vi "numbe_estimation.vi"(8 "桁数":i32=4, 11 "数値":i32) -> (3 "数値文字列":string)   [LabVIEW 2018]
panel:
  out "文字列":string
  out "配列":string[](array[string])
  out "10進数整数文字列":string
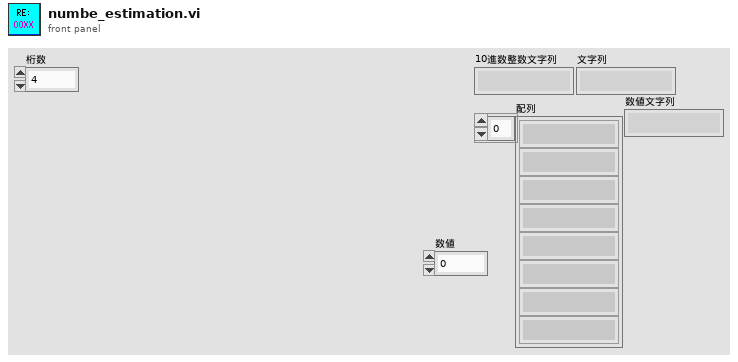
[diagram p1: front panel]
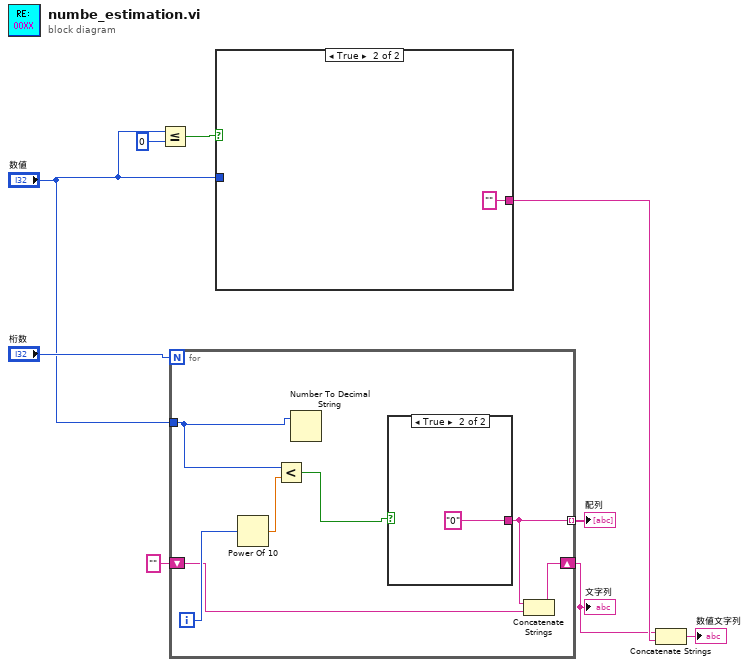
[diagram p0: block diagram]
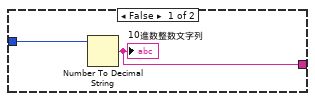
[diagram p2: hidden frame]
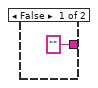
[diagram p3: hidden frame]
diagram:
  n1 = Less Or Equal?(x="数値", y=0) -> (x <= y?=w1:bool)
  n2 = for {
    N: "桁数" -> [_]
    tunnel: "数値" -> [w14]
    tunnel: [w12] -> w8 mode=indexing
    shift-right: [w10] -> w4
    shift-left: "" ("10進数整数文字列 2") -> [w11]
    i -> [w16]
    n3 = Power Of 10(x=w16) -> (10^x=w15:dbl)
    n4 = Less?(x=w14, y=w15) -> (x < y?=w13:bool)
    n5 = Number To Decimal String(number=w14) -> ()  [unwired: 1 in, 1 out]
    n6 = case shown="True" w13 {
      tunnel: ["" ("10進数整数文字列 2") "0" ("10進数整数文字列 2")] -> w12
      frame False {
      }
      frame True {
      }
    }
    n7 = Concatenate Strings(w12, w11) -> (w10:string)
  }
  "配列" <- w8
  "文字列" <- w4
  n8 = case shown="True" w1 {
    tunnel: [w20 ""] -> w6
    tunnel: "数値" -> [w19 _]
    frame False {
      n9 = Number To Decimal String(number=w19) -> (decimal integer string=w20:string)  [unwired: 1 in]
      "10進数整数文字列" <- w20
    }
    frame True {
    }
  }
  n10 = Concatenate Strings(w4, w6) -> (→"数値文字列":string)
